vi "Create Queue.vi"(8 "error in (no error)":errorcluster, 9 "Region":T1, 10 "Name":string, 11 "AWS Credentials":T2) -> (0 "error out":errorcluster, 3 "SQS":refnum<class "Queue.lvclass">)   [LabVIEW 2015, in "NI_AWS_SQS.lvlib" / "Queue.lvclass"]
doc: "Creates a new standard or FIFO queue or returns the URL of an existing queue. You can pass one or more attributes in the request. Keep the following caveats in mind:\n\nIf you don't specify the FifoQueue attribute, Amazon SQS creates a standard queue.\nNote\nYou can't change the queue type after you create it and you can't convert an existing standard queue into a FIFO queue. You must either create a new FIFO queue for your application or delete your existing standard queue and recreate it as a FIFO queue. For more information, see Moving From a Standard Queue to a FIFO Queue in the Amazon SQS Developer Guide.\nIf you don't provide a value for an attribute, the queue is created with the default value for the attribute.\nIf you delete a queue, you must wait at least 60 seconds before creating a queue with the same name.\nTo successfully create a new queue, you must provide a queue name that adheres to the limits related to queues and is unique within the scope of your queues.\n\nTo get the queue URL, use the GetQueueUrl action. GetQueueUrl requires only the QueueName parameter. be aware of existing queue names:\n\nIf you provide the name of an existing queue along with the exact names and values of all the queue's attributes, CreateQueue returns the queue URL for the existing queue.\nIf the queue name, attribute names, or attribute values don't match an existing queue, CreateQueue returns an error."
uses:
  Queue.lvclass
  Core/HTTP Request/AWS Credentials.ctl
  Core/HTTP Request/Region.ctl
  Core/HTTP Request/Request Options.ctl
  Core/HTTP Request/Name Value Pair.ctl
  Core/HTTP Request/Region handling.ctl
  Core/HTTP Request/URL formatting.ctl
  Core/HTTP Request/HTTP Request.lvclass/HTTP Request.ctl
  Queue.lvclass/Queue.ctl
  Core/HTTP Request/Write Credentials.vi
  Core/HTTP Request/Write Region.vi
  Core/HTTP Request/Write Service.vi
  Core/HTTP Request/Write Verify Server.vi
  Write Account Number.vi
  Write Name.vi
  Write URL.vi
  Core/HTTP Request/HTTP Request.lvclass
  XML Parsing/NI_XML Parsing.lvlib
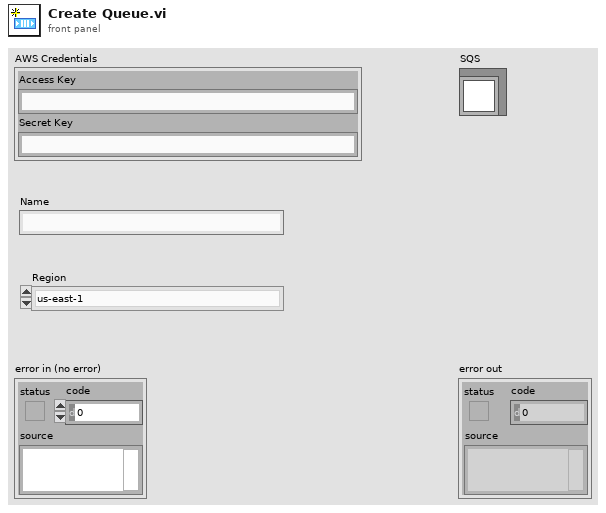
[diagram p1: front panel]
types:
  T1 = typedef "NI_AWS_Core.lvlib/HTTP Request.lvclass/Region.ctl" = enum16{"us-east-1", "us-east-2", "us-west-1", "us-west-2", "ap-northeast-1", "ap-northeast-2", "ap-southeast-1", "ap-southeast-2", "ca-central-1", "eu-central-1", "eu-west-1", "eu-west-2", "sa-east-1"}
  T2 = typedef "NI_AWS_Core.lvlib/HTTP Request.lvclass/AWS Credentials.ctl" = cluster{"Access Key":string, "Secret Key":string}
  T3 = typedef "NI_AWS_Core.lvlib/HTTP Request.lvclass/Name Value Pair.ctl" = cluster{"name":string, "value":string}
  T4 = typedef "NI_AWS_Core.lvlib/HTTP Request.lvclass/Request Options.ctl" = cluster{"request headers":T3[], "request parameters":T3[], "request body":string, "region handling":T5, "URL formatting":T6}
  T5 = typedef "NI_AWS_Core.lvlib/HTTP Request.lvclass/Region handling.ctl" = enum16{"use region everywhere", "use region (authentication only)", "use region (URL only)", "ignore region everwhere"}
  T6 = typedef "NI_AWS_Core.lvlib/HTTP Request.lvclass/URL formatting.ctl" = enum16{"region-", "region."}
  T7 = typedef "NI_AWS_Core.lvlib/HTTP Request.lvclass/Response.ctl" = cluster{"Headers":string, "Body":string}
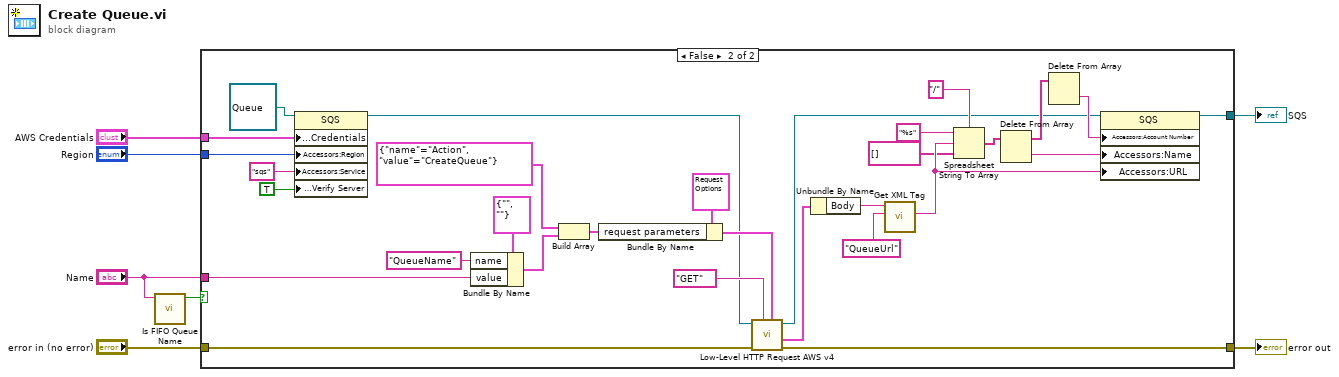
[diagram p0: block diagram]
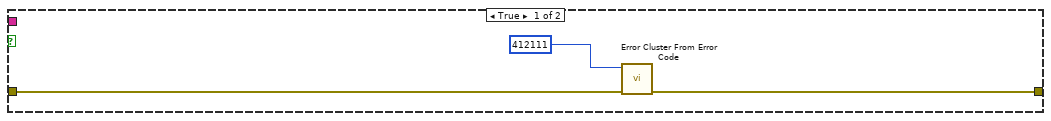
[diagram p2: hidden frame]
diagram:
  n1 = call "Is FIFO Queue Name.vi"("Name"="Name") -> ("FIFO Queue"=w1:bool)  [unwired: 10 in]
  n2 = case shown="False" w1 {
    tunnel: "AWS Credentials" -> [_ w40]
    tunnel: [w9 w39] -> w6
    tunnel: "error in (no error)" -> [w10 w38]
    tunnel: [_ w37] -> w4
    tunnel: "Region" -> [_ w36]
    tunnel: "Name" -> [_ w16]
    frame True {
      n3 = call <vilib>:"Error Cluster From Error Code.vi"("error in (no error)"=w10, "error code (0)"=412111) -> ("error out"=w9:errorcluster)  [unwired: 7 in]
    }
    frame False {
      n4 = property class="SQS"(reference=refnum<class "Queue.lvclass"> refnum ("NI_SQS.lvlib:SQS"), "Accessors:Credentials"=w40, "Accessors:Region"=w36, "Accessors:Service"="sqs" ("Service"), "Accessors:Verify Server"=TRUE ("Verify Server")) -> (reference out=w12:refnum<class "Queue.lvclass">)  [unwired: 1 in, 1 out]
      n5 = Bundle By Name(cluster=T3 {"name"="", "value"=""} ("element"), "name"="QueueName", "value"=w16) -> (w17:T3)
      n6 = Build Array(T3 {"name"="Action", "value"="CreateQueue"} ("Name Value Pair"), w17) -> (w21:T3[])
      n7 = Bundle By Name(cluster=T4 {"request headers"=[], "request parameters"=[{"name"="Action", "value"="ListQueues"}], "request body"="", "region handling"=enum."use region everywhere", "URL formatting"=enum."region."} ("Request Options"), "request parameters"=w21) -> (w13:T4)
      n8 = call "Low-Level HTTP Request AWS v4.vi"("Request Options"=w13, "HTTP-Verb"="GET", "error in (no error)"=w38, "AWS Core in"=w12) -> ("error out"=w39:errorcluster, "Response"=w15:T7, "AWS Core out"=w11:refnum<class "Queue.lvclass">)  [unwired: 4 in, 1 out]
      n9 = Unbundle By Name(w15) -> ("Body"=w22:string)
      n10 = call "Get XML Tag.vi"("Tag name"="QueueUrl", "XML String in"=w22) -> ("Tag value"=w30:string)  [unwired: 5 in, 4 out]
      n11 = Spreadsheet String To Array(delimiter (Tab)="/", format string="%s", spreadsheet string=w30, array type (2D Dbl)=string[] []) -> (array=w26:string[])
      n12 = Delete From Array(array=w26) -> (deleted portion=w25:string, array with subset deleted=w24:string[])  [unwired: 2 in]
      n13 = Delete From Array(array=w24) -> (deleted portion=w23:string)  [unwired: 2 in, 1 out]
      n14 = property class="SQS"(reference=w11, "Accessors:Account Number"=w23, "Accessors:Name"=w25, "Accessors:URL"=w30) -> (reference out=w37:refnum<class "Queue.lvclass">)  [unwired: 1 in, 1 out]
    }
  }
  "error out" <- w6
  "SQS" <- w4
